vi "LayerCluster_ValueChange.vi"(7 "Old Visibility?":bool, 8 "error in":errorcluster, 9 "Old name":string, 10 "CtlRef":refnum<vi>, 11 "Data in":T1={"Class"={"Ants"=refnum, "Layer"=refnum, "Templates"=refnum, "Icon"=refnum, "Glyph"=refnum, "Settings"=refnum, "Tools"=refnum, "History"=refnum}, "Ref"={"Add Layer"=refnum, "Remove Layer"=refnum, "Line Text"=[], "Body Text Spec"=refnum, "DNL_Font"=refnum, "glyph path str"=refnum, "templates path str"=refnum, "Arrow Up"=refnum, "Arrow Down"=refnum, "IE VI Ref"=refnum, "Glyphs tree"=refnum, "Templates tree"=refnum, "Layer Icon Text"=refnum, "Layer Template"=refnum, "Body Text"=refnum, "Search Templates"=refnum, "TextMarker"=refnum, "Tab Control"=refnum, "Search Glyphs"=refnum, "Line Color"=refnum, "DNL_Glyphs []"=refnum, "Fill Color"=refnum, "Tools"=refnum, "Icon"=refnum, "Preview"=refnum, "Ants"=refnum, "Terminals"=refnum, "menu reference"=refnum, "LayerNames"=[], "GlyphLoadAnimation"=refnum, "TemplateLoadAnimation"=refnum, "refreshGlyphs"=refnum, "refreshTemplates"=refnum}, "Support"={"AntsRect"={"left"=0, "top"=0, "right"=0, "bottom"=0}, "Mouse Move Coords"={"Horizontal"=0, "Vertical"=0}, "Mouse Down Coords"={"Horizontal"=0, "Vertical"=0}, "Temp Coord"={"Horizontal"=0, "Vertical"=0}, "Action"=enum."Default", "Edge Color"=4914962, "Fill Color"=16860, "Mouse Down?"=FALSE, "Draft Mode?"=FALSE, "Temp Icon"=bytes[3102], "CTRL Pressed"=FALSE, "Move Selection?"=FALSE, "AntsRect Orig"={"left"=0, "top"=0, "right"=0, "bottom"=0}, "Text"="", "TM Set?"=FALSE, "Mouse inside icon?"=FALSE, "Tool (old value)"=0, "Pencil Move Color"=0, "Swap Colors?"=FALSE, "Shift pressed?"=FALSE}}) -> (0 "error out":errorcluster, 3 "Data out":T1={"Class"={"Ants"=refnum, "Layer"=refnum, "Templates"=refnum, "Icon"=refnum, "Glyph"=refnum, "Settings"=refnum, "Tools"=refnum, "History"=refnum}, "Ref"={"Add Layer"=refnum, "Remove Layer"=refnum, "Line Text"=[], "Body Text Spec"=refnum, "DNL_Font"=refnum, "glyph path str"=refnum, "templates path str"=refnum, "Arrow Up"=refnum, "Arrow Down"=refnum, "IE VI Ref"=refnum, "Glyphs tree"=refnum, "Templates tree"=refnum, "Layer Icon Text"=refnum, "Layer Template"=refnum, "Body Text"=refnum, "Search Templates"=refnum, "TextMarker"=refnum, "Tab Control"=refnum, "Search Glyphs"=refnum, "Line Color"=refnum, "DNL_Glyphs []"=refnum, "Fill Color"=refnum, "Tools"=refnum, "Icon"=refnum, "Preview"=refnum, "Ants"=refnum, "Terminals"=refnum, "menu reference"=refnum, "LayerNames"=[], "GlyphLoadAnimation"=refnum, "TemplateLoadAnimation"=refnum, "refreshGlyphs"=refnum, "refreshTemplates"=refnum}, "Support"={"AntsRect"={"left"=0, "top"=0, "right"=0, "bottom"=0}, "Mouse Move Coords"={"Horizontal"=0, "Vertical"=0}, "Mouse Down Coords"={"Horizontal"=0, "Vertical"=0}, "Temp Coord"={"Horizontal"=0, "Vertical"=0}, "Action"=enum."Default", "Edge Color"=4914962, "Fill Color"=16860, "Mouse Down?"=FALSE, "Draft Mode?"=FALSE, "Temp Icon"=bytes[3102], "CTRL Pressed"=FALSE, "Move Selection?"=FALSE, "AntsRect Orig"={"left"=0, "top"=0, "right"=0, "bottom"=0}, "Text"="", "TM Set?"=FALSE, "Mouse inside icon?"=FALSE, "Tool (old value)"=0, "Pencil Move Color"=0, "Swap Colors?"=FALSE, "Shift pressed?"=FALSE}})   [LabVIEW 2020]
uses:
  Class/Ants/Ants.lvclass
  Class/FakedArray/FakedArray.lvclass
  vi.lib/LabVIEW Icon API/lv_icon/Classes/Icon/Icon.lvclass
  Class/Icon Library/Glyph.lvclass
  Class/Settings/Settings.lvclass
  Class/Tools/Tools Paint.lvclass
  History/History/History.lvclass
  vi.lib/LabVIEW Icon API/lv_icon/Classes/Layer/Layer.lvclass
  Controls/SupportClass_Action.ctl
  History/History.lvlib
  vi.lib/LabVIEW Icon API/lv_icon/Controls/Layer.ctl
  <vilib>/Utility/miscctls.llb/LVPoint32TypeDef.ctl
  vi.lib/LabVIEW Icon API/lv_icon/Controls/IEColor.ctl
  Controls/Support Cluster.ctl
  lv_icon.lvlib
  Controls/References Cluster.ctl
  Controls/IE Classes.ctl
  Controls/Global Data.ctl
panel:
  in  "?":T8={"LayerIcon"=bytes[3102], "LayerName"="", "Opacity"=100, "Visibility?"=TRUE} {"Opacity" scale=0.0..100.0}
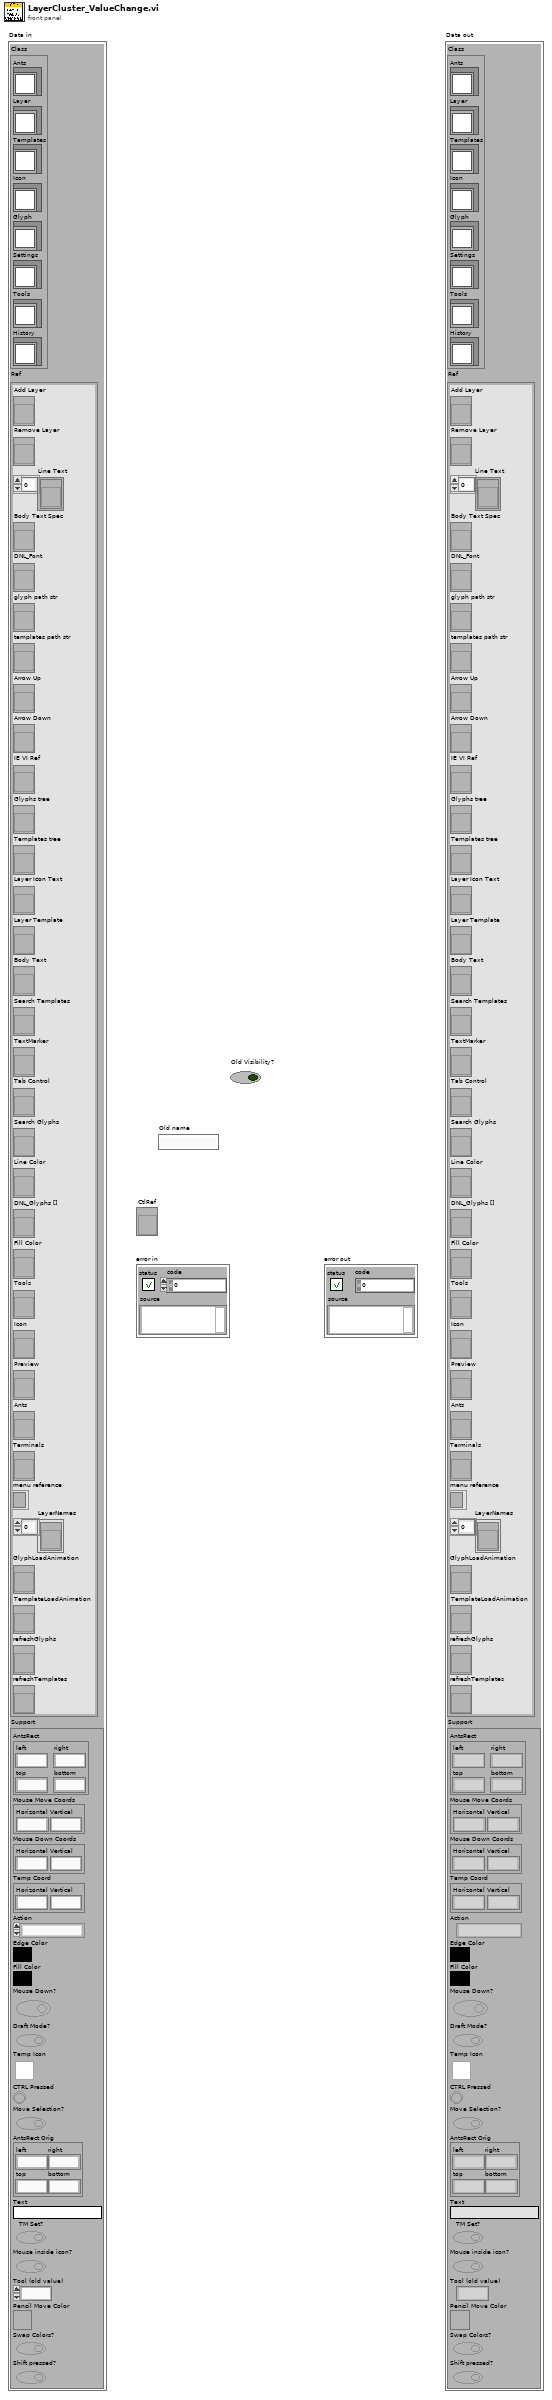
[diagram p1: front panel]
types:
  T1 = typedef "lv_icon.lvlib/Global Data.ctl" = cluster{"Class":T2, "Ref":T3, "Support":T4}
  T2 = typedef "lv_icon.lvlib/IE Classes.ctl" = cluster{"Ants":refnum<class "Ants.lvclass">, "Layer":refnum<class "FakedArray.lvclass">, "Templates":refnum<class "FakedArray.lvclass">, "Icon":refnum<class "Icon.lvclass">, "Glyph":refnum<class "Glyph.lvclass">, "Settings":refnum<class "Settings.lvclass">, "Tools":refnum<class "Tools Paint.lvclass">, "History":refnum<class "History.lvclass">}
  T3 = typedef "lv_icon.lvlib/References Cluster.ctl" = cluster{"Add Layer":refnum<vi>, "Remove Layer":refnum<vi>, "Line Text":refnum<vi>[], "Body Text Spec":refnum<vi>, "DNL_Font":refnum<vi>, "glyph path str":refnum<vi>, "templates path str":refnum<vi>, "Arrow Up":refnum<vi>, "Arrow Down":refnum<vi>, "IE VI Ref":refnum<vi>, "Glyphs tree":refnum<vi>, "Templates tree":refnum<vi>, "Layer Icon Text":refnum<vi>, "Layer Template":refnum<vi>, "Body Text":refnum<vi>, "Search Templates":refnum<vi>, "TextMarker":refnum<vi>, "Tab Control":refnum<vi>, "Search Glyphs":refnum<vi>, "Line Color":refnum<vi>, "DNL_Glyphs []":refnum<vi>, "Fill Color":refnum<vi>, "Tools":refnum<vi>, "Icon":refnum<vi>, "Preview":refnum<vi>, "Ants":refnum<vi>, "Terminals":refnum<vi>, "menu reference":refnum<k9>, "LayerNames":refnum<vi>[], "GlyphLoadAnimation":refnum<vi>, "TemplateLoadAnimation":refnum<vi>, "refreshGlyphs":refnum<vi>, "refreshTemplates":refnum<vi>}
  T4 = typedef "lv_icon.lvlib/Support Cluster.ctl" = cluster{"AntsRect":cluster{"left":i16, "top":i16, "right":i16, "bottom":i16}, "Mouse Move Coords":T5, "Mouse Down Coords":T5, "Temp Coord":T5, "Action":T6, "Edge Color":T7, "Fill Color":T7, "Mouse Down?":bool, "Draft Mode?":bool, "Temp Icon":picture, "CTRL Pressed":bool, "Move Selection?":bool, "AntsRect Orig":cluster{"left":i16, "top":i16, "right":i16, "bottom":i16}, "Text":string, "TM Set?":bool, "Mouse inside icon?":bool, "Tool (old value)":u32, "Pencil Move Color":u32, "Swap Colors?":bool, "Shift pressed?":bool}
  T5 = typedef "LVPoint32TypeDef.ctl" = cluster{"Horizontal":i32, "Vertical":i32}
  T6 = typedef "SupportClass_Action.ctl" = enum16{"Default", "Move Selection", "Glyph Library", "Tool"}
  T7 = typedef "IEColor.ctl" = u32
  T8 = typedef "Layer.ctl" = cluster{"LayerIcon":picture, "LayerName":string, "Opacity":u8, "Visibility?":bool}
  T9 = cluster{"Horizontal":i32, "Vertical":i32, "Vertical 2":i32, "Vertical 3":i32}
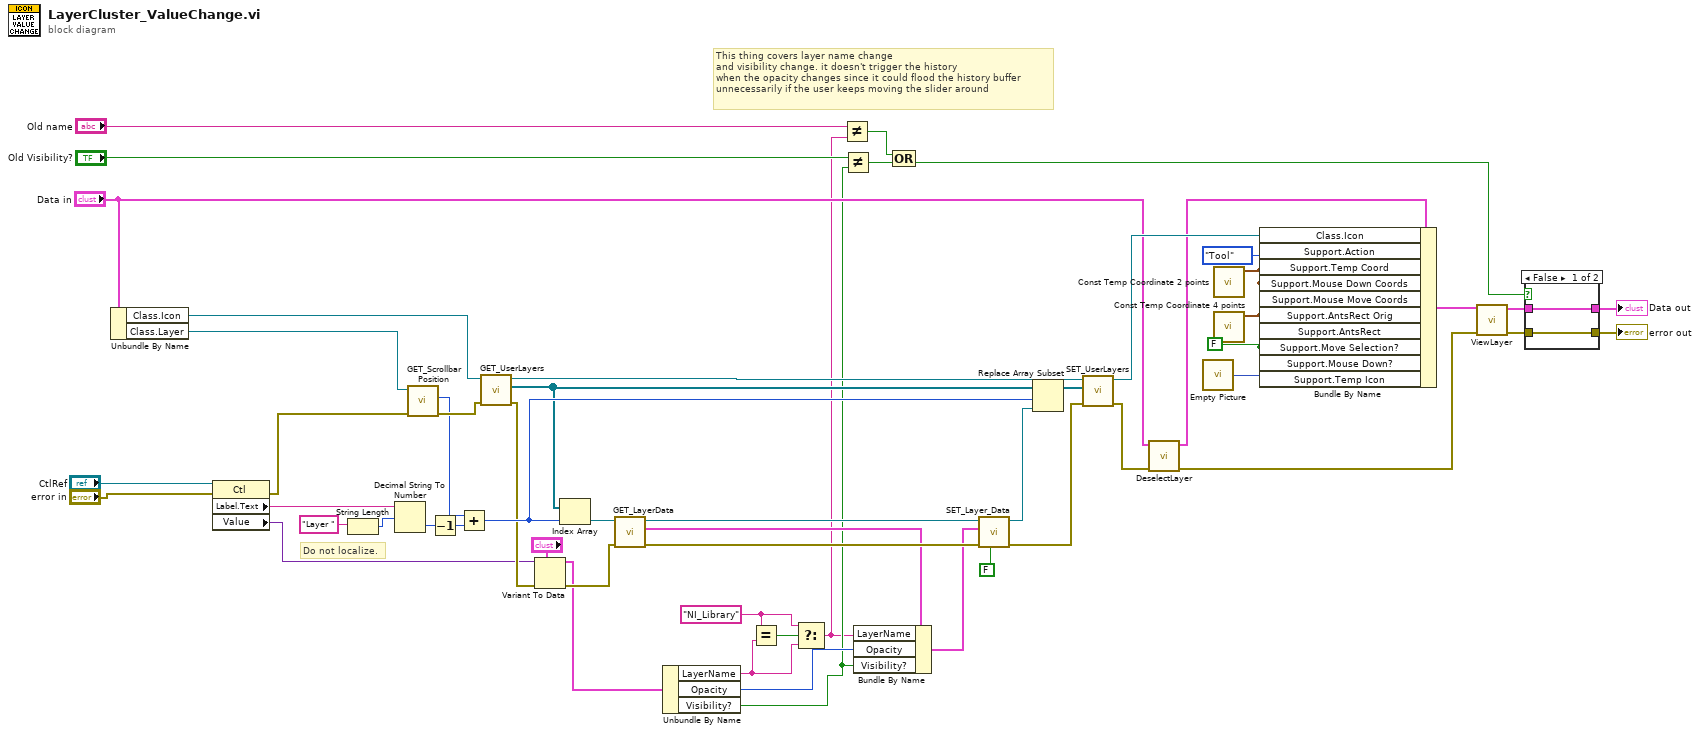
[diagram p0: block diagram]
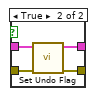
[diagram p2: hidden frame]
diagram:
  w15 = "NI_Library" ("x")
  w34 = FALSE ("Mouse Down?")
  # "This thing covers layer name change\nand visibility change. it doesn't trigger the history\nwhen the opacity changes since it could flood the history buffer\nunnecessarily if the user keeps moving the slider around"
  # "Do not localize."
  n1 = Unbundle By Name("Data in") -> ("Class.Icon"=w40:refnum<class "Icon.lvclass">, "Class.Layer"=w39:refnum<class "FakedArray.lvclass">)
  n2 = property class="Ctl"(reference="CtlRef", error in="error in") -> (error out=w30:errorcluster, "Label.Text"=w45:string, "Value"=w49:variant)  [unwired: 1 out]
  n3 = String Length(string="Layer ") -> (length=w41:i32)
  n4 = Decimal String To Number(string=w45, offset=w41) -> (number=w47:i32)  [unwired: 2 out]
  n5 = call-dynamic "GET_Scrollbar Position.vi"("error in (no error)"=w30, "FakedArray.lvclass in"=w39) -> ("error out"=w50:errorcluster, "Scrollbar Position"=w48:i32)  [unwired: 8 out]
  n6 = Decrement(x=w47) -> (x-1=w46:i32)
  n7 = Add(x=w48, y=w46) -> (x+y=w55:i32)
  n8 = call-dynamic "GET_UserLayers.vi"("error in (no error)"=w50, "Icon.lvclass in"=w40) -> ("error out"=w52:errorcluster, "All Layers"=w54:refnum<class "Layer.lvclass">[], "Icon.lvclass out"=w51:refnum<class "Icon.lvclass">)  [unwired: 7 out]
  n9 = Variant To Data(error in=w52, type="?", Variant=w49) -> (data=w14:T8, error out=w23:errorcluster)
  n10 = Index Array(array=w54, index=w55) -> (element=w25:refnum<class "Layer.lvclass">)
  n11 = call-dynamic "GET_LayerData.vi"("error in (no error)"=w23, "Layer.lvclass in"=w25) -> ("error out"=w22:errorcluster, "Data"=w16:T8, "Layer.lvclass out"=w24:refnum<class "Layer.lvclass">)  [unwired: 7 out]
  n12 = Unbundle By Name(w14) -> ("LayerName"=w11:string, "Opacity"=w13:u8, "Visibility?"=w9:bool)
  n13 = Equal?(x=w15, y=w11) -> (x = y?=w12:bool)
  n14 = Select(t=w15, s=w12, f=w11) -> (s? t:f=w7:string)
  n15 = Not Equal?(x="Old name", y=w7) -> (x != y?=w5:bool)
  n16 = Not Equal?(x="Old Visibility?", y=w9) -> (x != y?=w8:bool)
  n17 = Bundle By Name(cluster=w16, "LayerName"=w7, "Opacity"=w13, "Visibility?"=w9) -> (w17:T8)
  n18 = Compound Arithmetic op=OR(w5, w8) -> (w1:bool)
  n19 = call-dynamic "SET_Layer_Data.vi"("Layer Tab Value Change? (F)"=FALSE, "error in (no error)"=w22, "Data"=w17, "Layer.lvclass in"=w24) -> ("error out"=w21:errorcluster, "Layer.lvclass out"=w20:refnum<class "Layer.lvclass">)  [unwired: 6 out]
  n20 = Replace Array Subset(array=w54, new element=w20, index=w55) -> (w18:refnum<class "Layer.lvclass">[])
  n21 = call-dynamic "SET_UserLayers.vi"("error in (no error)"=w21, "Layers"=w18, "Icon.lvclass in"=w51) -> ("error out"=w29:errorcluster, "Icon.lvclass out"=w38:refnum<class "Icon.lvclass">)  [unwired: 7 in]
  n22 = call "DeselectLayer.vi"("error in (no error)"=w29, "Data in"="Data in") -> ("error out"=w27:errorcluster, "Data out"=w31:T1)  [unwired: 8 out]
  n23 = call "Empty Picture"() -> ("empty picture"=w33:picture)
  n24 = call "Const Temp Coordinate 2 points.vi"() -> ("Const Temp Coordinate"=w36:T5)  [unwired: 11 out]
  n25 = call "Const Temp Coordinate 4 points.vi"() -> ("Const Temp Coordinate"=w35:T9)  [unwired: 11 out]
  n26 = Bundle By Name(cluster=w31, "Class.Icon"=w38, "Support.Action"=SupportClass_Action."Tool" ("Action"), "Support.Temp Coord"=w36, "Support.Mouse Down Coords"=w36, "Support.Mouse Move Coords"=w36, "Support.AntsRect Orig"=w35, "Support.AntsRect"=w35, "Support.Move Selection?"=w34, "Support.Mouse Down?"=w34, "Support.Temp Icon"=w33) -> (w28:T1)
  n27 = call "ViewLayer.vi"("error in (no error)"=w27, "Data in"=w28) -> ("error out"=w26:errorcluster, "Data out"=w3:T1)  [unwired: 3 in, 5 out]
  n28 = case shown="False" w1 {
    tunnel: w26 -> [w56 w61]
    tunnel: [w56 w60] -> w4
    tunnel: w3 -> [w57 w59]
    tunnel: [w57 w58] -> w2
    frame False {
    }
    frame True {
      n29 = call "Set Undo Flag.vi"("error in"=w61, "Data in"=w59) -> ("error out"=w60:errorcluster, "Data out"=w58:T1)  [unwired: 8 in]
    }
  }
  "error out" <- w4
  "Data out" <- w2
